vi "Test Asserts.vi"(8 "error in (no error)":errorcluster) -> (0 "error out":errorcluster)   [LabVIEW 2020]
uses:
  tests/test-lvlib/test-lvlib.lvlib
  Test/Test.lvclass
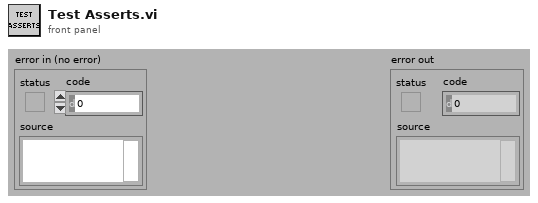
[diagram p1: front panel]
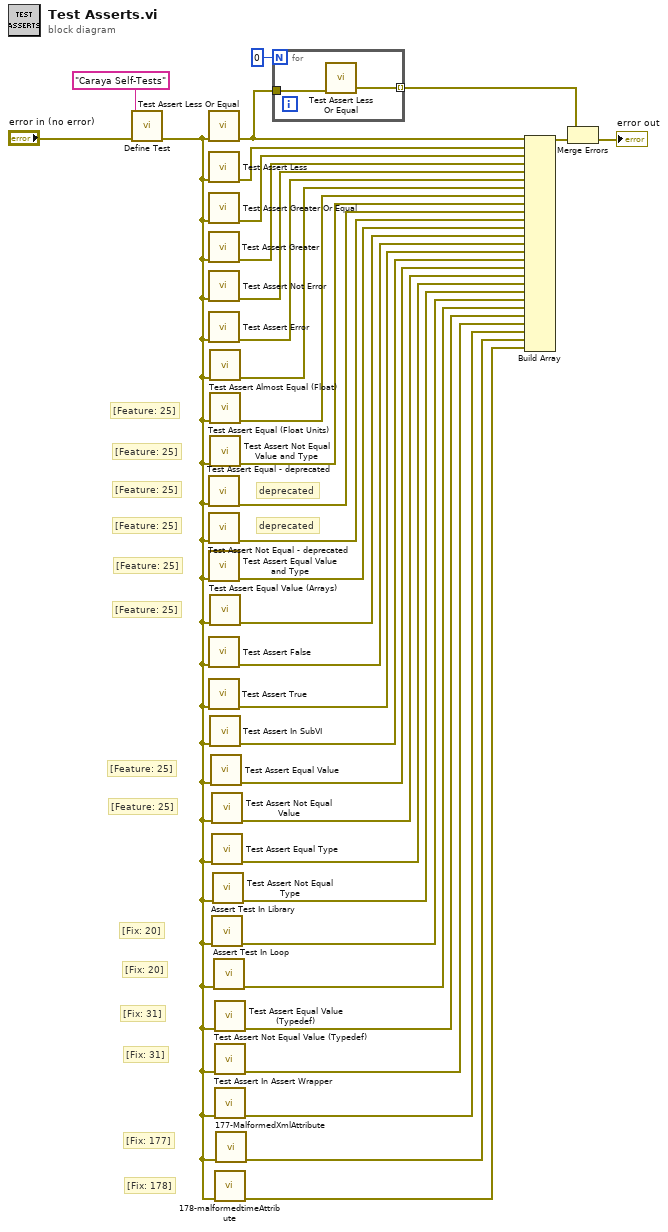
[diagram p0: block diagram]
diagram:
  # "[Fix: 178]"
  # "[Fix: 177]"
  # "[Fix: 31]"
  # "[Fix: 31]"
  # "[Fix: 20]"
  # "[Fix: 20]"
  # "[Feature: 25]"
  # "[Feature: 25]"
  # "[Feature: 25]"
  # "[Feature: 25]"
  # "[Feature: 25]"
  # "[Feature: 25]"
  # "[Feature: 25]"
  # "[Feature: 25]"
  # "deprecated"
  # "deprecated"
  n1 = call "Define Test.vi"("error in (no error)"="error in (no error)", "Label (VI Title)"="Caraya Self-Tests") -> ("error out"=w2:errorcluster)  [unwired: 8 in, 1 out]
  n2 = call "Test Assert Less Or Equal.vi"("error in (no error)"=w2) -> ("error out"=w7:errorcluster)  [unwired: 10 in]
  n3 = call "Test Assert Less.vi"("error in (no error)"=w2) -> ("error out"=w34:errorcluster)  [unwired: 10 in]
  n4 = call "Test Assert Greater Or Equal.vi"("error in (no error)"=w2) -> ("error out"=w33:errorcluster)  [unwired: 10 in]
  n5 = call "Test Assert Greater.vi"("error in (no error)"=w2) -> ("error out"=w32:errorcluster)  [unwired: 10 in]
  n6 = call "Test Assert Not Error.vi"("error in (no error)"=w2) -> ("error out"=w31:errorcluster)  [unwired: 10 in]
  n7 = call "Test Assert Error.vi"("error in (no error)"=w2) -> ("error out"=w30:errorcluster)  [unwired: 10 in]
  n8 = call "Test Assert Equal - deprecated.vi"("error in (no error)"=w2) -> ("error out"=w20:errorcluster)  [unwired: 10 in]
  n9 = call "Test Assert Not Equal - deprecated.vi"("error in (no error)"=w2) -> ("error out"=w29:errorcluster)  [unwired: 10 in]
  n10 = call "Test Assert Equal Value and Type.vi"("error in (no error)"=w2) -> ("error out"=w28:errorcluster)  [unwired: 10 in]
  n11 = call "Test Assert False.vi"("error in (no error)"=w2) -> ("error out"=w27:errorcluster)  [unwired: 10 in]
  n12 = call "Test Assert True.vi"("error in (no error)"=w2) -> ("error out"=w26:errorcluster)  [unwired: 10 in]
  n13 = call "Test Assert Almost Equal (Float).vi"("error in (no error)"=w2) -> ("error out"=w19:errorcluster)  [unwired: 10 in]
  n14 = call "Test Assert Equal (Float Units).vi"("error in (no error)"=w2) -> ("error out"=w16:errorcluster)  [unwired: 10 in]
  n15 = call "Test Assert Not Equal Value and Type.vi"("error in (no error)"=w2) -> ("error out"=w18:errorcluster)  [unwired: 10 in]
  n16 = call "Test Assert Equal Value (Arrays).vi"("error in (no error)"=w2) -> ("error out"=w17:errorcluster)  [unwired: 10 in]
  n17 = call "Test Assert In SubVI.vi"("error in (no error)"=w2) -> ("error out"=w23:errorcluster)  [unwired: 10 in]
  n18 = call "Test Assert Equal Value.vi"("error in (no error)"=w2) -> ("error out"=w22:errorcluster)  [unwired: 10 in]
  n19 = call "Test Assert Not Equal Value.vi"("error in (no error)"=w2) -> ("error out"=w21:errorcluster)  [unwired: 10 in]
  n20 = call "Test Assert Equal Type.vi"("error in (no error)"=w2) -> ("error out"=w15:errorcluster)  [unwired: 10 in]
  n21 = call "Assert Test In Library.vi"("error in (no error)"=w2) -> ("error out"=w13:errorcluster)  [unwired: 10 in]
  n22 = call "Test Assert Not Equal Type.vi"("error in (no error)"=w2) -> ("error out"=w14:errorcluster)  [unwired: 10 in]
  n23 = call "Assert Test In Loop.vi"("error in (no error)"=w2) -> ("error out"=w12:errorcluster)  [unwired: 10 in]
  n24 = call "Test Assert Equal Value (Typedef).vi"("error in"=w2) -> ("error out"=w11:errorcluster)  [unwired: 10 in]
  n25 = call "Test Assert Not Equal Value (Typedef).vi"("error in (no error)"=w2) -> ("error out"=w10:errorcluster)  [unwired: 10 in]
  n26 = call "Test Assert In Assert Wrapper.vi"("error in (no error)"=w2) -> ("error out"=w4:errorcluster)  [unwired: 10 in]
  n27 = call "178-malformedtimeAttribute.vi"("error in"=w2) -> ("error out"=w1:errorcluster)  [unwired: 10 in]
  n28 = call "177-MalformedXmlAttribute.vi"("error in"=w2) -> ("error out"=w3:errorcluster)  [unwired: 10 in]
  n29 = for {
    N: 0 -> [_]
    tunnel: w7 -> [w36]
    tunnel: [w35] -> w6 mode=indexing
    n30 = call "Test Assert Less Or Equal.vi"("error in (no error)"=w36) -> ("error out"=w35:errorcluster)  [unwired: 10 in]
  }
  n31 = Build Array(w7, w34, w33, w32, w31, w30, w19, w16, w18, w20, w29, w28, w17, w27, w26, w23, w22, w21, w15, w14, w13, w12, w11, w10, w4, w3, w1) -> (w25:errorcluster[])
  n32 = Merge Errors(w6, w25) -> (→"error out":errorcluster)
